vi "Update RPC Client Method Controls.vi"(5 "Library":refnum<vi>, 6 "RPC Method Parameters":T1, 8 "error in (no error)":errorcluster, 11 "VI in":refnum<vi>) -> (0 "error out":errorcluster, 3 "VI out":refnum<vi>)   [LabVIEW 2019, in "gRPC Template Creation Utility.lvlib"]
uses:
  gRPC Template Creation Utility.lvlib
  TypeDefs/RPC Method Parameters.ctl
  <vilib>/Utility/traverseref.llb/TRef TravTarget.ctl
  63320222-a0c5-46f2-a668-ff10f55be25f.vi
  108da764-e401-4abd-a40a-091b83fc4494.vi
  <vilib>/Comparison/Equal/Equal Functor/Equal Functor.lvclass
  <vilib>/Utility/traverseref.llb/VI Scripting - Traverse.lvlib
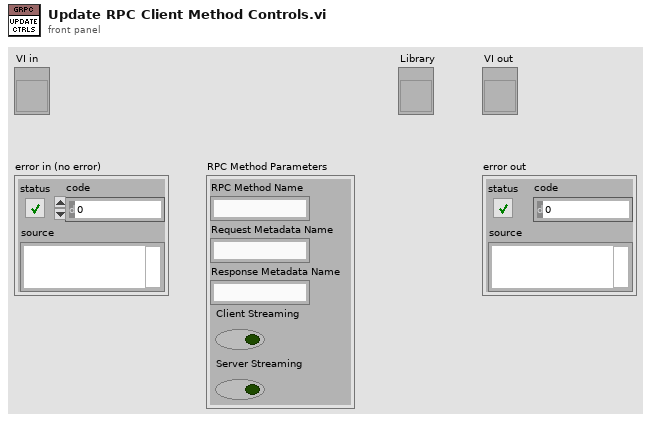
[diagram p1: front panel]
types:
  T1 = typedef "gRPC Template Creation Utility.lvlib/RPC Method Parameters.ctl" = cluster{"RPC Method Name":string, "Request Metadata Name":string, "Response Metadata Name":string, "Client Streaming":bool, "Server Streaming":bool}
  T2 = typedef "TRef TravTarget.ctl" = enum16{"FP", "BD", "Other"}
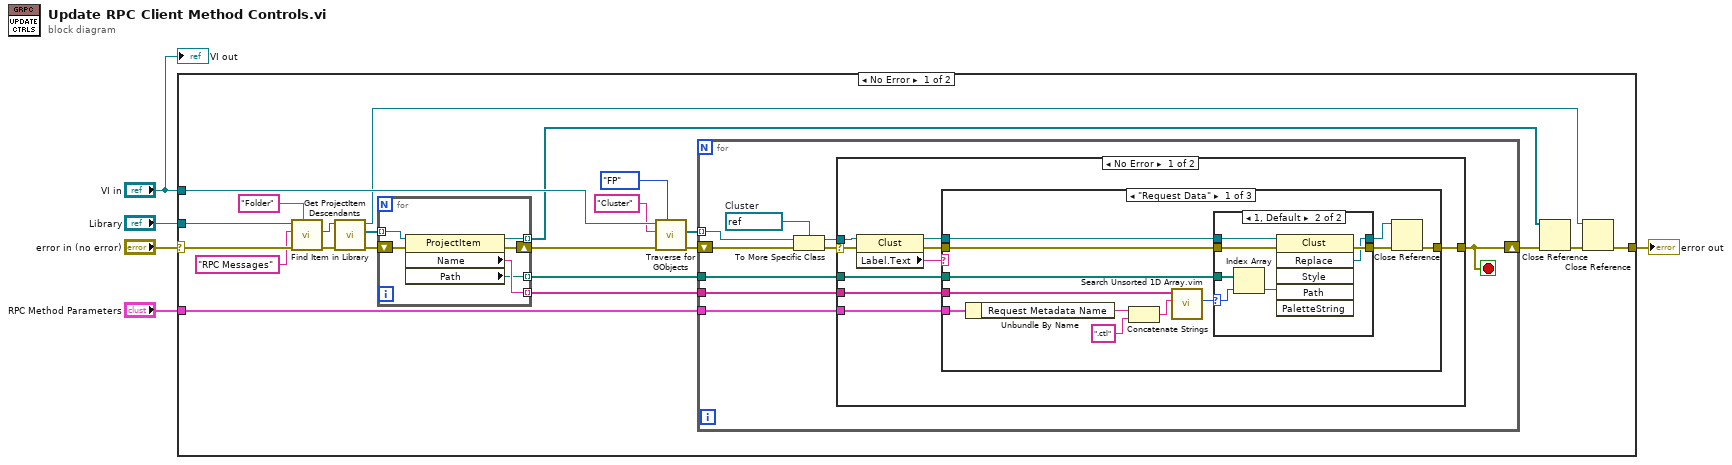
[diagram p0: block diagram]
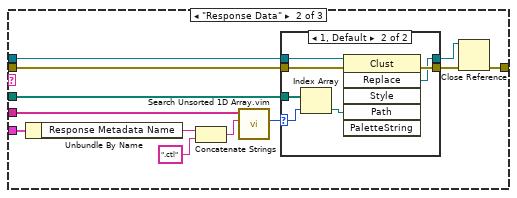
[diagram p3: hidden frame]
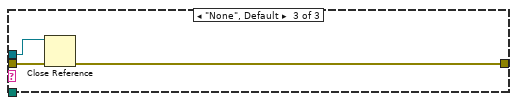
[diagram p5: hidden frame]
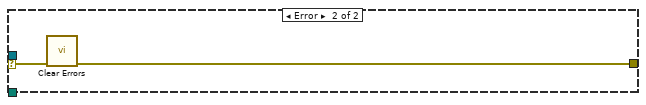
[diagram p6: hidden frame]
diagram:
  n1 = case shown="No Error" "error in (no error)" {
    selector: "error in (no error)" -> [w26 w99]
    tunnel: [w27 w99] -> w5
    tunnel: "VI in" -> [w25 _]
    tunnel: "Library" -> [w24 _]
    tunnel: "RPC Method Parameters" -> [w23 _]
    frame No Error {
      n2 = call "Find Item in Library.vi"("Item Type"="Folder", "error in (no error)"=w26, "Item Name"="RPC Messages", "Library item in"=w24) -> ("error out"=w17:errorcluster, "Project Item (Library Item)"=w16:refnum<vi>)  [unwired: 4 in, 2 out]
      n3 = call "Get ProjectItem Descendants.vi"("error in (no error)"=w17, "ProjectItem in"=w16) -> ("error out"=w13:errorcluster, "All Descendents"=w18:refnum<vi>[], "ProjectItem out"=w11:refnum<vi>)  [unwired: 7 in]
      n4 = for {
        tunnel: w18 -> [w33] mode=indexing
        tunnel: [w32] -> w10 mode=indexing
        tunnel: [w31] -> w9 mode=indexing
        shift-right: [w29] -> w12
        shift-left: w13 -> [w30]
        tunnel: [w28] -> w8 mode=indexing
        n5 = property class="ProjectItem"(reference=w33, error in=w30) -> (reference out=w31:refnum<vi>, error out=w29:errorcluster, "Name"=w32:string, "Path"=w28:path)
      }
      n6 = call <vilib>:"Traverse for GObjects.vi"("Traverse Target"=TRef_TravTarget."FP", "error in (no error)"=w12, "Class Name"="Cluster", "VI Refnum"=w25) -> ("error out"=w20:errorcluster, "References"=w19:refnum<vi>[])  [unwired: 4 in, 2 out]
      n7 = for {
        tunnel: w19 -> [w35] mode=indexing
        shift-right: [w34] -> w6
        shift-left: w20 -> [w41]
        tunnel: w23 -> [w38]
        tunnel: w10 -> [w37]
        tunnel: w8 -> [w36]
        stop <- w34 stop-if-true
        w42 = refnum<vi> refnum  # Cluster
        n8 = To More Specific Class(target class=w42, reference=w35, error in=w41) -> (specific class reference=w40:refnum<vi>, error out=w39:errorcluster)
        n9 = case shown="No Error" w39 {
          selector: w39 -> [w50 w98]
          tunnel: w40 -> [w51 _]
          tunnel: [w46 w97] -> w34
          tunnel: w38 -> [w45 _]
          tunnel: w37 -> [w44 _]
          tunnel: w36 -> [w43 _]
          frame No Error {
            n10 = property class="Clust"(reference=w51, error in=w50) -> (reference out=w48:refnum<vi>, error out=w47:errorcluster, "Label.Text"=w49:string)
            n11 = case shown="\"Request Data\"" w49 {
              tunnel: w48 -> [w56 w77 w94]
              tunnel: w47 -> [w55 w76 w96]
              tunnel: [w53 w73 w95] -> w46
              tunnel: w45 -> [w63 w84 _]
              tunnel: w44 -> [w60 w81 _]
              tunnel: w43 -> [w58 w79 _]
              frame "Request Data" {
                n12 = Unbundle By Name(w63) -> ("Request Metadata Name"=w62:string)
                n13 = Concatenate Strings(w62, ".ctl" ("string")) -> (w59:string)
                n14 = call "Search Unsorted 1D Array.vim"("element"=w59, "unsorted 1D array"=w60) -> ("index of element"=w57:i32)  [unwired: 9 in]
                n15 = case shown="1, Default" w57 {
                  selector: w57 -> [_ w71]
                  tunnel: w58 -> [_ w72]
                  tunnel: w56 -> [w64 w70]
                  tunnel: w55 -> [w65 w69]
                  tunnel: [w65 w67] -> w54
                  tunnel: [w64 w66] -> w52
                  frame -1 {
                  }
                  frame 1, Default {
                    n16 = Index Array(array=w72, index=w71) -> (element=w68:path)
                    n17 = invoke class="Clust" method="Replace"(reference=w70, error in=w69, "Path"=w68) -> (error out=w67:errorcluster, "Replace"=w66:refnum<vi>)  [unwired: 3 in, 4 out]
                  }
                }
                n18 = Close Reference(reference=w52, error in (no error)=w54) -> (error out=w53:errorcluster)
              }
              frame "Response Data" {
                n19 = Unbundle By Name(w84) -> ("Response Metadata Name"=w83:string)
                n20 = Concatenate Strings(w83, ".ctl" ("string")) -> (w80:string)
                n21 = call "Search Unsorted 1D Array.vim"("element"=w80, "unsorted 1D array"=w81) -> ("index of element"=w78:i32)  [unwired: 9 in]
                n22 = case shown="1, Default" w78 {
                  selector: w78 -> [_ w92]
                  tunnel: w79 -> [_ w93]
                  tunnel: w77 -> [w85 w91]
                  tunnel: [w85 w87] -> w74
                  tunnel: w76 -> [w86 w90]
                  tunnel: [w86 w89] -> w75
                  frame -1 {
                  }
                  frame 1, Default {
                    n23 = Index Array(array=w93, index=w92) -> (element=w88:path)
                    n24 = invoke class="Clust" method="Replace"(reference=w91, error in=w90, "Path"=w88) -> (error out=w89:errorcluster, "Replace"=w87:refnum<vi>)  [unwired: 3 in, 4 out]
                  }
                }
                n25 = Close Reference(reference=w74, error in (no error)=w75) -> (error out=w73:errorcluster)
              }
              frame "None", Default {
                n26 = Close Reference(reference=w94, error in (no error)=w96) -> (error out=w95:errorcluster)
              }
            }
          }
          frame Error {
            n27 = call <vilib>:"Clear Errors.vi"("error in (no error)"=w98) -> ("error out"=w97:errorcluster)  [unwired: 5 in, 1 out]
          }
        }
      }
      n28 = Close Reference(reference=w9, error in (no error)=w6) -> (error out=w7:errorcluster)
      n29 = Close Reference(reference=w11, error in (no error)=w7) -> (error out=w27:errorcluster)
    }
    frame Error {
    }
  }
  "error out" <- w5
  "VI out" <- "VI in"
